vi "Stop.vi"(1 "Engine":refnum<k7>) -> (0 "Error Out":errorcluster)   [LabVIEW 2021, in "Seq Edit Quick Drop.lvlib"]
uses:
  Seq Edit Quick Drop.lvlib
  Message.ctl
  Command.ctl
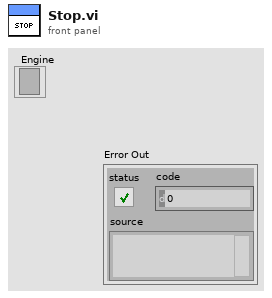
[diagram p1: front panel]
types:
  T1 = typedef "Seq Edit Quick Drop.lvlib/Message.ctl" = cluster{"cmd":T2, "data":variant}
  T2 = typedef "Seq Edit Quick Drop.lvlib/Command.ctl" = enum16{"Init", "Get Application Manager", "Shortcut Activated", "Display Tools", "Tool Selected", "Timeout", "Error", "Close"}
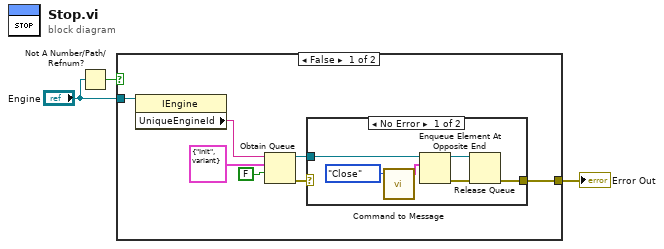
[diagram p0: block diagram]
diagram:
  n1 = Not A Number/Path/Refnum?(number/path/refnum="Engine") -> (NaN/Path/Refnum?=w2:bool)
  n2 = case shown="False" w2 {
    tunnel: "Engine" -> [w10 _]
    tunnel: [w5 _] -> w1
    frame False {
      n3 = property class="IEngine"(reference=w10) -> ("UniqueEngineId"=w4:string)  [unwired: 1 in, 2 out]
      n4 = Obtain Queue(name (unnamed)=w4, element data type=T1 {"cmd"=enum."Init", "data"=variant} ("msg"), create if not found? (T)=FALSE) -> (queue out=w7:refnum<queue>, error out=w6:errorcluster)  [unwired: 2 in, 1 out]
      n5 = case shown="No Error" w6 {
        selector: w6 -> [_ w17]
        tunnel: w7 -> [w14 _]
        tunnel: [w12 w17] -> w5
        frame No Error {
          n6 = call "Command to Message.vi"("cmd"=Command."Close") -> ("msg"=w15:T1)  [unwired: 4 in]
          n7 = Enqueue Element At Opposite End(queue=w14, element=w15) -> (queue out=w11:refnum<queue>, error out=w13:errorcluster)  [unwired: 2 in, 1 out]
          n8 = Release Queue(queue=w11, error in (no error)=w13) -> (error out=w12:errorcluster)  [unwired: 1 in, 2 out]
        }
        frame Error {
        }
      }
    }
    frame True {
    }
  }
  "Error Out" <- w1
